vi "Running State.vi"(1 "value in (F)":bool, 2 "action (get)":enum16{"Set", "Get"}(ring)=enum."Get") -> (0 "value out":bool)   [LabVIEW 2018, in "GLog.lvlib" / "Registry.lvlib"]
uses:
  Registry.lvlib
panel:
  # "Connector Pane"
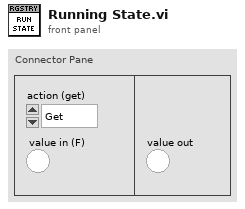
[diagram p1: front panel]
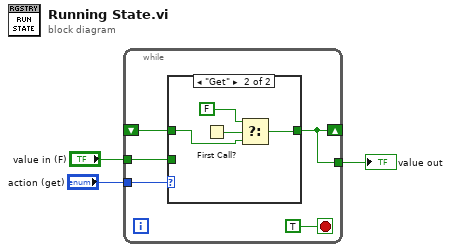
[diagram p0: block diagram]
diagram:
  n1 = while {
    tunnel: "action (get)" -> [w8]
    shift-right: [w6] -> _
    shift-left: _ -> [w7]
    tunnel: [w6] -> w2
    tunnel: "value in (F)" -> [w5]
    stop <- TRUE stop-if-true
    n2 = case shown="\"Get\"" w8 {
      tunnel: [w9 w11] -> w6
      tunnel: w7 -> [_ w10]
      tunnel: w5 -> [w9 _]
      frame "Set" {
      }
      frame "Get" {
        n3 = First Call?() -> (First Call?: T/F=w13:bool)
        n4 = Select(t=FALSE, s=w13, f=w10) -> (s? t:f=w11:bool)
      }
    }
  }
  "value out" <- w2
